vi "TP_Example.vi"() -> ()   [LabVIEW 2020]
panel:
  out "Q 6":bool
  out "ET 6":i32
  out "Q 5":bool
  out "ET 5":i32
  out "ET 4":i32
  out "Q 4":bool
  in  "Trigger":bool
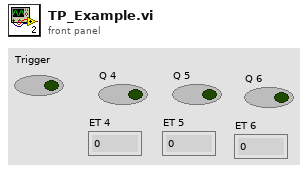
[diagram p1: front panel]
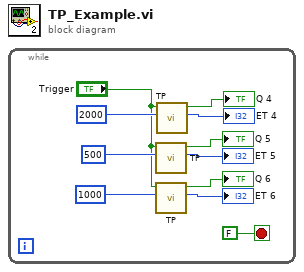
[diagram p0: block diagram]
diagram:
  n1 = while {
    stop <- FALSE stop-if-true
    n2 = call "TP.vi"("Time"=500, "Trigger"="Trigger") -> ("ET 4"=→"ET 5":i32, "Q 4"=→"Q 5":bool)  [unwired: 8 in]
    n3 = call "TP.vi"("Time"=1000, "Trigger"="Trigger") -> ("ET 4"=→"ET 6":i32, "Q 4"=→"Q 6":bool)  [unwired: 8 in]
    n4 = call "TP.vi"("Time"=2000, "Trigger"="Trigger") -> ("ET 4"=→"ET 4":i32, "Q 4"=→"Q 4":bool)  [unwired: 8 in]
  }
